vi "Calculating_motion.vi"(8 "Error IN":errorcluster={"status"=FALSE, "code"=0, "source"="5000"}, 10 "Motion sequence":T1, 11 "Constants IN":T3) -> (0 "Error OUT":errorcluster, 2 "Output":T2, 3 "Constants OUT":T3)   [LabVIEW 2019]
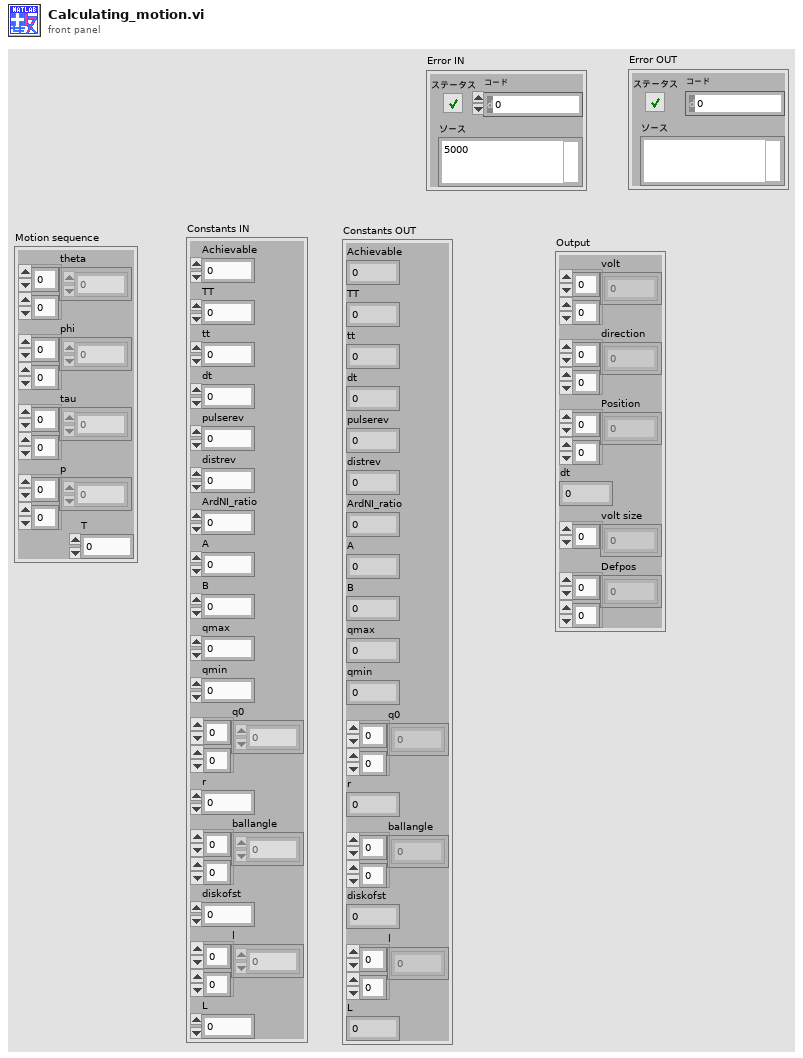
[diagram p1: front panel]
types:
  T1 = cluster{"theta":dbl[][], "phi":dbl[][], "tau":dbl[][], "p":dbl[][], "T":dbl}
  T2 = cluster{"volt":dbl[][], "direction":dbl[][], "Position":dbl[][], "dt":dbl, "volt size":i32[], "Defpos":dbl[][]}
  T3 = cluster{"Achievable":dbl, "TT":dbl, "tt":dbl, "dt":dbl, "pulserev":dbl, "distrev":dbl, "ArdNI_ratio":dbl, "A":dbl, "B":dbl, "qmax":dbl, "qmin":dbl, "q0":dbl[][], "r":dbl, "ballangle":dbl[][], "diskofst":dbl, "l":dbl[][], "L":dbl}
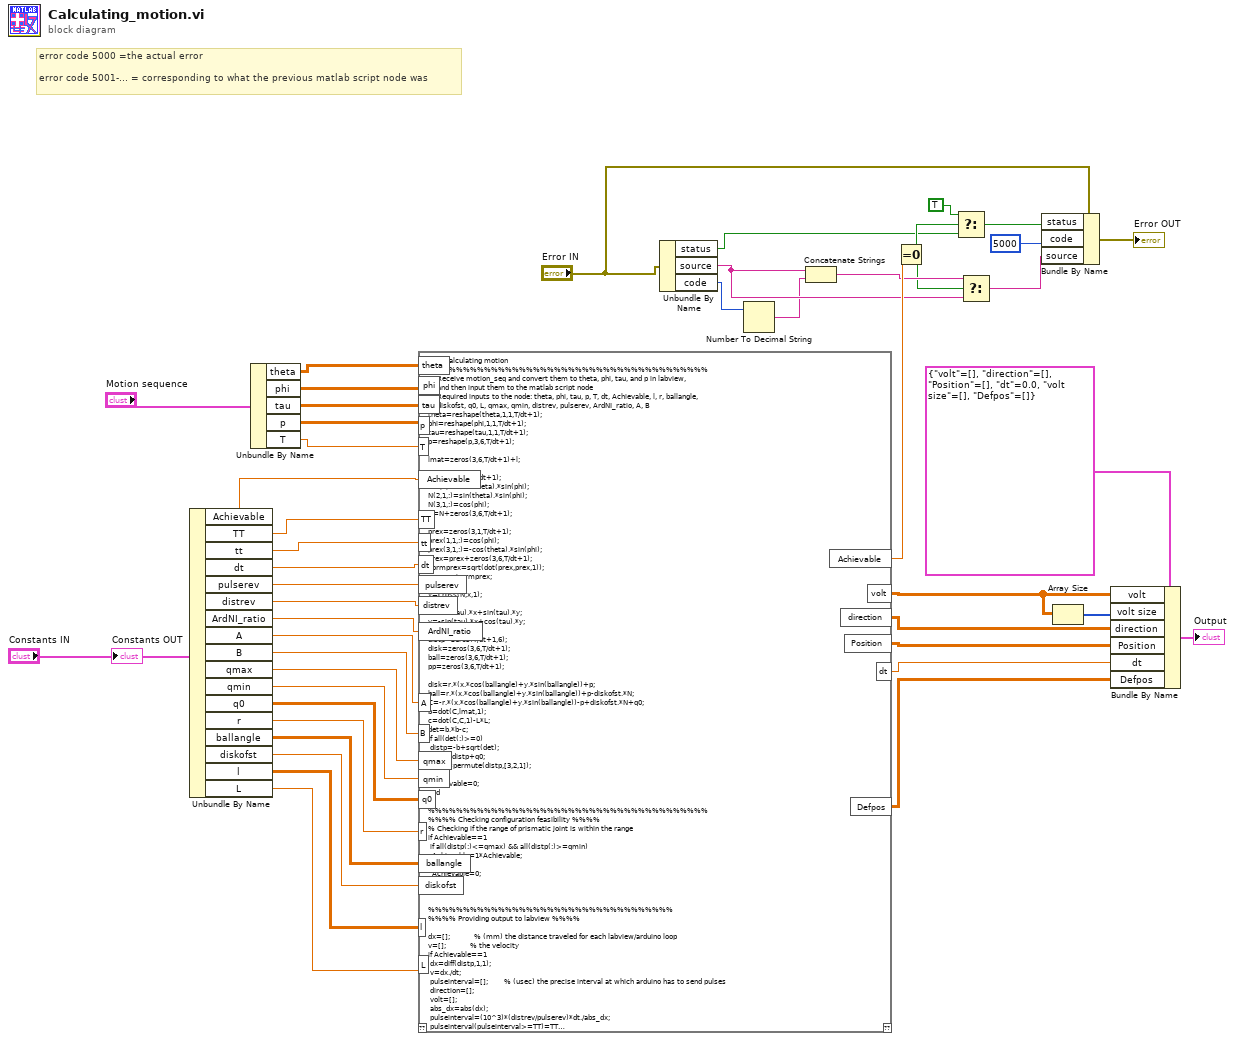
[diagram p0: block diagram]
diagram:
  # "error code 5000 =the actual error\n\nerror code 5001-... = corresponding to what the previous matlab script node was"
  n1 = Unbundle By Name("Constants IN") -> ("Achievable"=w44:dbl, "TT"=w43:dbl, "tt"=w42:dbl, "dt"=w41:dbl, "pulserev"=w40:dbl, "distrev"=w39:dbl, "ArdNI_ratio"=w38:dbl, "A"=w37:dbl, "B"=w36:dbl, "qmax"=w35:dbl, "qmin"=w34:dbl, "q0"=w33:dbl[][], "r"=w32:dbl, "ballangle"=w31:dbl[][], "diskofst"=w30:dbl, "l"=w29:dbl[][], "L"=w28:dbl)
  n2 = Unbundle By Name("Motion sequence") -> ("theta"=w14:dbl[][], "phi"=w13:dbl[][], "tau"=w12:dbl[][], "p"=w11:dbl[][], "T"=w1:dbl)
  n3 = script code="%% Calculating motion\n%%%%%%%%%%%%%%%%%%%%%%%%%%%%%%%%%%%%%%%%\n% Receive motion_seq and convert them to theta, phi, tau, and p in labview,\n% and then input them to the matlab script node\n% Required inputs to the node: theta, phi, tau, p, T, dt, Achievable, l, r, ballangle,\n% diskofst, q0, L, qmax, qmin, distrev, pulserev, ArdNI_ratio, A, B\ntheta=reshape(theta,1,1,T/dt+1);\nphi=reshape(phi,1,1,T/dt+1);\ntau=reshape(tau,1,1,T/dt+1);\np=reshape(p,3,6,T/dt+1);\n\nlmat=zeros(3,6,T/dt+1)+l;\n\nN=zeros(3,1,T/dt+1);\nN(1,1,:)=cos(theta).*sin(phi);\nN(2,1,:)=sin(theta).*sin(phi);\nN(3,1,:)=cos(phi);\nN=N+zeros(3,6,T/dt+1);\n\nprex=zeros(3,1,T/dt+1);\nprex(1,1,:)=cos(phi);\nprex(3,1,:)=-cos(theta).*sin(phi);\nprex=prex+zeros(3,6,T/dt+1);\nnormprex=sqrt(dot(prex,prex,1));\nx=prex./normprex;\n\ny=cross(N,x,1);\n\nx=cos(tau).*x+sin(tau).*y;\ny=-sin(tau).*x+cos(tau).*y;\n\ndistp=zeros(T/dt+1,6);\ndisk=zeros(3,6,T/dt+1);\nball=zeros(3,6,T/dt+1);\npp=zeros(3,6,T/dt+1);\n\ndisk=r.*(x.*cos(ballangle)+y.*sin(ballangle))+p;\nball=r.*(x.*cos(ballangle)+y.*sin(ballangle))+p-diskofst.*N;\nC=-r.*(x.*cos(ballangle)+y.*sin(ballangle))-p+diskofst.*N+q0;\nb=dot(C,lmat,1);\nc=dot(C,C,1)-L*L;\ndet=b.*b-c;\nif all(det(:)>=0)\n\tdistp=-b+sqrt(det);\n\tpp=l.*distp+q0;\n\tdistp=permute(distp,[3,2,1]);\nelse\n\tAchievable=0;\nend\n\n%%%%%%%%%%%%%%%%%%%%%%%%%%%%%%%%%%%%%%%%\n%%%% Checking configuration feasibility %%%%\n% Checking if the range of prismatic joint is within the range\nif Achievable==1\n\tif all(distp(:)<=qmax) && all(distp(:)>=qmin)\n\t\tAchievable=1*Achievable;\n\telse\n\t\tAchievable=0;\n\tend\nend\n\n%%%%%%%%%%%%%%%%%%%%%%%%%%%%%%%%%%%\n%%%% Providing output to labview %%%%\n\ndx=[];\t\t\t\t\t\t\t\t\t\t\t\t% (mm) the distance traveled for each labview/arduino loop\nv=[];\t\t\t\t\t\t\t\t\t\t\t\t% the velocity\nif Achievable==1\n\tdx=diff(distp,1,1);\n\tv=dx./dt;\n\tpulseinterval=[];\t\t\t\t\t\t\t\t% (usec) the precise interval at which arduino has to send pulses\n\tdirection=[];\n\tvolt=[];\n\tabs_dx=abs(dx);\n\tpulseinterval=(10^3)*(distrev/pulserev)*dt./abs_dx;\n\tpulseinterval(pulseinterval>=TT)=TT;\t\t\t% Making sure that pulseinterval does not exceed TT\n\tif all(pulseinterval(:)>=tt)\n\t\tAchievable=1*Achievable;\n\telse\n\t\tAchievable=0;\t\t\t\t\t\t\t\t% Making sure that the speed is achievable (pulseinterval is less than or equal to tt)\n\tend\n\tvolt=(5/(1024*ArdNI_ratio))*((B./pulseinterval)-A);\n\tdirection=sign(dx);\n\tdirection=(1/2)*(direction+1);\nend\n\nDefpos=distp(1,:);\t\t\t\t\t\t\t\t% This is where the prismatic joints start their movement. So the prismatic joints have to be manually set to these precise values\nAdjDefpos=Defpos-9.206;\n\n\n%%%% Position relative to the initial position %%%%\nPosition=distp;\n\n% max_tt=min(pulseinterval,[],\"all\");\n\n% Total_pulse_count=sum(abs_dx./(distrev/pulserev),1);"("TT"=w43, "tt"=w42, "dt"=w41, "pulserev"=w40, "distrev"=w39, "ArdNI_ratio"=w38, "A"=w37, "B"=w36, "qmax"=w35, "qmin"=w34, "q0"=w33, "r"=w32, "ballangle"=w31, "diskofst"=w30, "l"=w29, "L"=w28, "Achievable"=w44, "theta"=w14, "phi"=w13, "tau"=w12, "p"=w11, "T"=w1) -> ("Achievable"=w27:dbl, "volt"=w7:dbl[][], "direction"=w9:dbl[][], "Position"=w8:dbl[][], "Defpos"=w4:dbl[][], "dt"=w5:dbl)  [unwired: 1 in, 1 out]
  n4 = Unbundle By Name("Error IN") -> ("status"=w15:bool, "source"=w24:string, "code"=w26:i32)
  n5 = Number To Decimal String(number=w26) -> (decimal integer string=w16:string)  [unwired: 1 in]
  n6 = Concatenate Strings(w24, w16) -> (w25:string)
  n7 = Equal To 0?(x=w27) -> (x = 0?=w21:bool)
  n8 = Select(t=TRUE ("status"), s=w21, f=w15) -> (s? t:f=w19:bool)
  n9 = Select(t=w25, s=w21, f=w24) -> (s? t:f=w23:string)
  n10 = Bundle By Name(cluster="Error IN", "status"=w19, "code"=5000, "source"=w23) -> (→"Error OUT":errorcluster)
  n11 = Array Size(array=w7) -> (size(s)=w6:i32[])
  n12 = Bundle By Name(cluster=T2 {"volt"=[], "direction"=[], "Position"=[], "dt"=0.0, "volt size"=[], "Defpos"=[]}, "volt"=w7, "volt size"=w6, "direction"=w9, "Position"=w8, "dt"=w5, "Defpos"=w4) -> (→"Output":T2)
  "Constants OUT" <- "Constants IN"
